vi "FuncVI-Moment.vi"(5 "InstanceRef":T2, 9 "arg list":T1[](array[typedef]) {"num" format="%.2f"}) -> (0 "error out":bool, 3 "result":T1 {"num" format="%.2f"})   [LabVIEW 2021]
doc: "::: CalcExpress Toolkit :::\nCopyright (c) 2000-2026 Konstantin Shifershteyn. All rights reserved."
uses:
  cetypes.llb/CalcExpress Function Argument Info.ctl
  cetypes.llb/CalcExpress Instance RefNum.ctl
  <vilib>/Analysis/NI_AALPro.lvlib
panel:
  in  "max arg num":i32=2
  in  "min arg num":i32=2
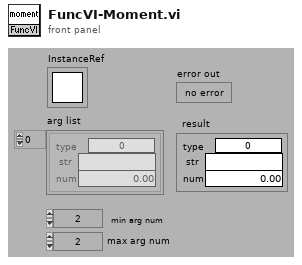
[diagram p1: front panel]
types:
  T1 = typedef "CalcExpress Function Argument Info.ctl" = cluster{"type":u32, "str":string, "num":dbl}
  T2 = typedef "CalcExpress Instance RefNum.ctl" = refnum<k1>
  T3 = enum32{"String", "DBL Number", "identifier", "1D Array of DBL", "2D Array of DBL", "CDB Number", "1D Array of CDB", "2D Array of CDB", "1D Array of String", "2D Array of String", "Unknown data type"}
  T4 = cluster{"use this constant to specify a predefined type":enum32{"String", "DBL Number", "identifier", "1D Array of DBL", "2D Array of DBL", "CDB Number", "1D Array of CDB", "2D Array of CDB", "1D Array of String", "2D Array of String", "Unknown data type"}, string, "moment":dbl}
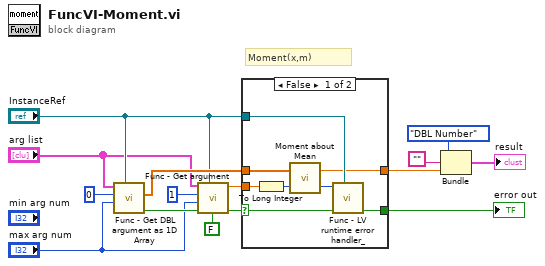
[diagram p0: block diagram]
diagram:
  # "Moment(x,m)"
  n1 = call "Func - Get DBL argument as 1D Array.vi"("InstanceRef"="InstanceRef", "max arg num"="max arg num", "arg idx"=0, "arg list"="arg list") -> ("error out"=w8:bool, "1D data"=w15:dbl[])  [unwired: 4 in, 2 out]
  n2 = call "Func - Get argument.vi"("ena NonNum? (F)"=FALSE, "InstanceRef"="InstanceRef", "error in"=w8, "max arg num"="max arg num", "arg idx"=1, "arg list"="arg list") -> ("error out"=w7:bool, "num"=w2:dbl)  [unwired: 2 out]
  n3 = case shown="False" w7 {
    selector: w7 -> [w23 w24]
    tunnel: w15 -> [w18 _]
    tunnel: [w19 _] -> w9
    tunnel: [w22 w24] -> w13
    tunnel: "InstanceRef" -> [w21 _]
    tunnel: w2 -> [w17 _]
    frame False {
      n4 = To Long Integer(number=w17) -> (32bit integer=w16:i32)
      n5 = call <vilib>:"Moment about Mean.vi"("order"=w16, "X"=w18) -> ("error"=w20:i32, "moment"=w19:dbl)
      n6 = call "Func - LV runtime error handler_.vi"("InstanceRef"=w21, "error in"=w23, "LabVIEW error code"=w20) -> ("error out"=w22:bool)  [unwired: 8 in]
    }
    frame True {
    }
  }
  "error out" <- w13
  n7 = Bundle("use this constant to specify a predefined type"=T3."DBL Number", "", "moment"=w9) -> (→"result":T4)  [unwired: 1 in]
